vi "Actor.vi"(4 "Async Elements":refnum<class "Async Elements.lvclass">, 7 "Actor in":refnum<class "Actor.lvclass">) -> (0 "Error out":errorcluster, 5 "Actor out":refnum<class "Actor.lvclass">)   [LabVIEW 2020, in "jettl.lvlib"]
uses:
  jettl.lvlib
  Actor/Actor.lvclass
  Async Elements/Async Elements.lvclass
  Stopped jettl Msg/Stopped/Tell Child.vi
  Stopped jettl Msg/Stopped/Tell Parent.vi
  Stopped jettl Msg/Stopped/Stopped.lvlib
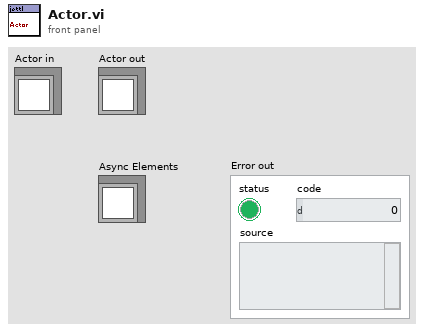
[diagram p1: front panel]
types:
  T1 = enum32{"Invalid", "Standard", "Closed", "Hidden", "Minimized", "Maximized"}
  T2 = typedef "jettl.lvlib/Child UIDs.ctl" = set{string}
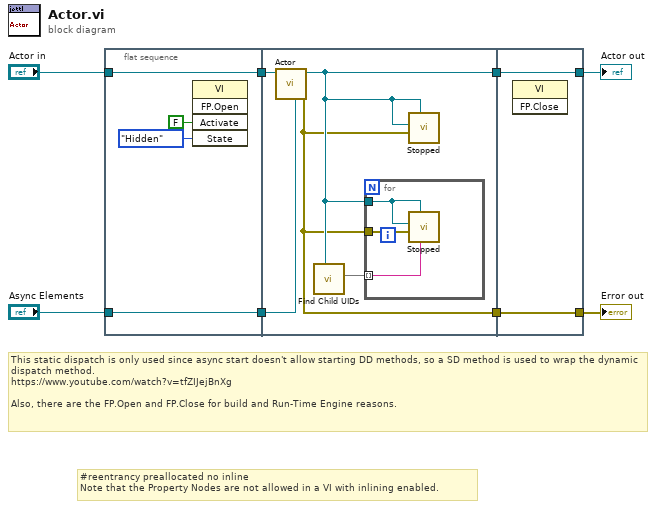
[diagram p0: block diagram]
diagram:
  # "#reentrancy preallocated no inline\nNote that the Property Nodes are not allowed in a VI with inlining enabled."
  # "This static dispatch is only used since async start doesn't allow starting DD methods, so a SD method is used to wrap the dynamic dispatch method.\nhttps://www.youtube.com/watch?v=tfZIJejBnXg\n\nAlso, there are the FP.Open and FP.Close for build and Run-Time Engine reasons."
  n1 = flat-sequence {
    tunnel: "Actor in" -> [w12]
    tunnel: [w12] -> w7
    tunnel: [w11] -> w6
    tunnel: "Async Elements" -> [w11]
    tunnel: w7 -> [w17]
    tunnel: w6 -> [w16]
    tunnel: [w13] -> w3
    tunnel: [w14] -> w2
    tunnel: [w22] -> w4
    tunnel: w3 -> [w22]
    tunnel: w2 -> [w21]
    tunnel: [w21] -> w1
    frame #0 {
      n2 = invoke class="VI" method="FP.Open"("Activate"=FALSE ("Activate?"), "State"=T1."Hidden") -> ()  [unwired: 3 in, 5 out]
    }
    frame #1 {
      n3 = call-dynamic "Actor.vi"("Async Elements"=w16, "Actor in"=w17) -> ("Error out"=w13:errorcluster, "Actor out"=w14:refnum<class "Actor.lvclass">)  [unwired: 8 in]
      n4 = call "Find Child UIDs.vi"("Actor in"=w14) -> ("Child UIDs"=w15:T2)  [unwired: 10 in]
      n5 = for {
        tunnel: w14 -> [w20]
        tunnel: w15 -> [w18] mode=indexing
        tunnel: w13 -> [w19]
        n6 = call-poly "Stopped.vi"("UID"=w18, "Actor in"=w20, "Error"=w19, "Actor"=w20) -> ()  [unwired: 6 in, 2 out]
      }
      n7 = call-poly "Stopped.vi"("Actor in"=w14, "Error"=w13, "Actor"=w14) -> ()  [unwired: 7 in, 2 out]
    }
    frame #2 {
      n8 = invoke class="VI" method="FP.Close"() -> ()  [unwired: 3 in, 3 out]
    }
  }
  "Actor out" <- w1
  "Error out" <- w4
